vi "CreateCompatibleBitmap Wrapper Template.vi"(0 "hdc":u64, 5 "cx":i32, 7 "cy":i32, 11 "error in":errorcluster) -> (4 "HBITMAP":u64, 15 "error out":errorcluster)   [LabVIEW 2020]
doc: "Creates a cx by cy bitmap compatible with the device context hdc through gdi32.dll CreateCompatibleBitmap (stdcall, called in any thread). Pass the SCREEN DC, not a fresh memory DC, or the bitmap is monochrome. Delete it with gdi32 DeleteObject.vi. When error in carries an error the DLL is not called. Generated by tools\\Build Win32 Wrappers.vi - do not edit by hand, rebuild it."
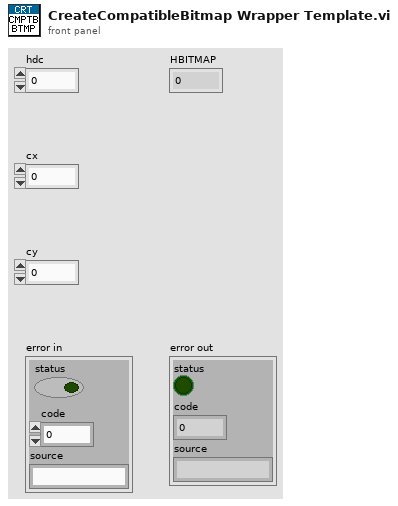
[diagram p1: front panel]
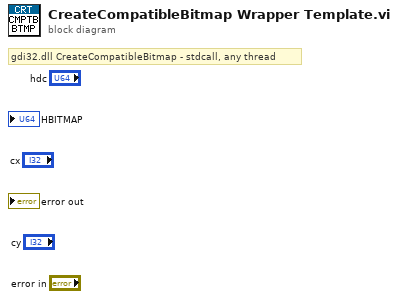
[diagram p0: block diagram]
diagram:
  # "gdi32.dll CreateCompatibleBitmap - stdcall, any thread"
